vi "Sample.vi"(8 "Error In":errorcluster caption="错误输入", 10 "基本信息":T1={"USB Port"="COM1", "采集间隔(s)"=0.5, "压力设备选择"=TRUE}) -> (0 "Error Out":errorcluster caption="错误输出", 2 "Data":dbl[](array[numeric]))   [LabVIEW 2026, in "UI-压力.lvlib" / "Acquisition.lvlib"]
uses:
  Acquisition.lvlib
  Supports/Device Info.ctl
  <vilib>/Analysis/baseanly.llb/Mean (DBL).vi
  <vilib>/Analysis/NI_AALBase.lvlib
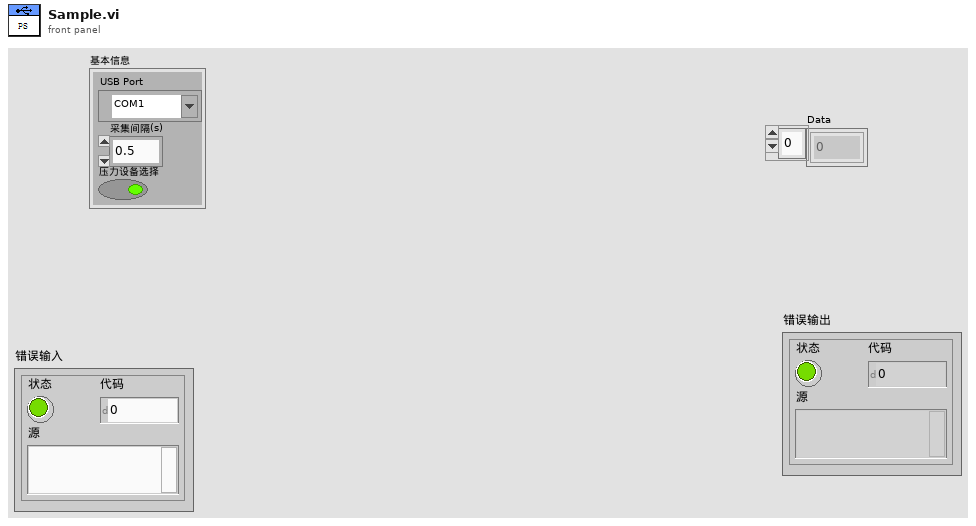
[diagram p1: front panel]
types:
  T1 = typedef "UI-压力.lvlib/Device Info.ctl" = cluster{"USB Port":refnum<visa-resource-name>, "采集间隔(s)":dbl, "压力设备选择":bool}
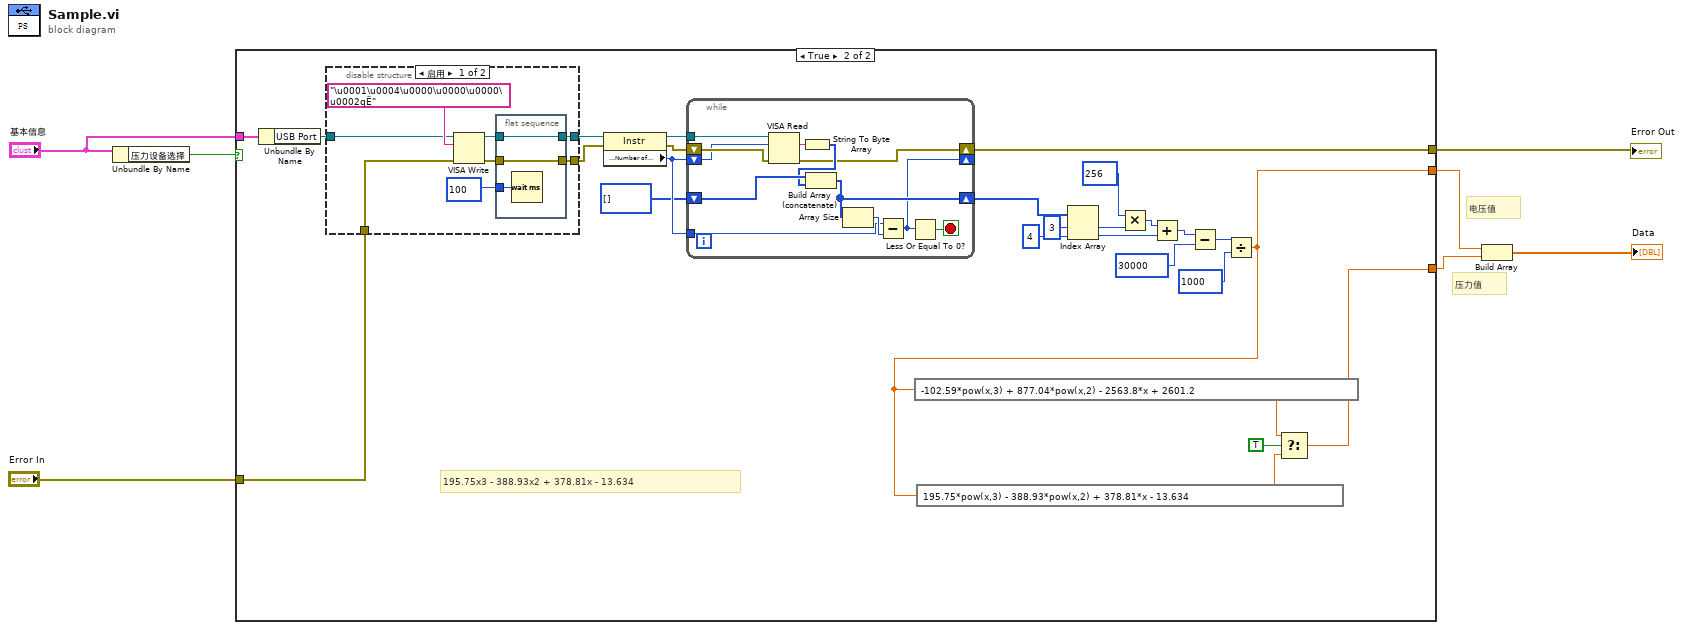
[diagram p0: block diagram]
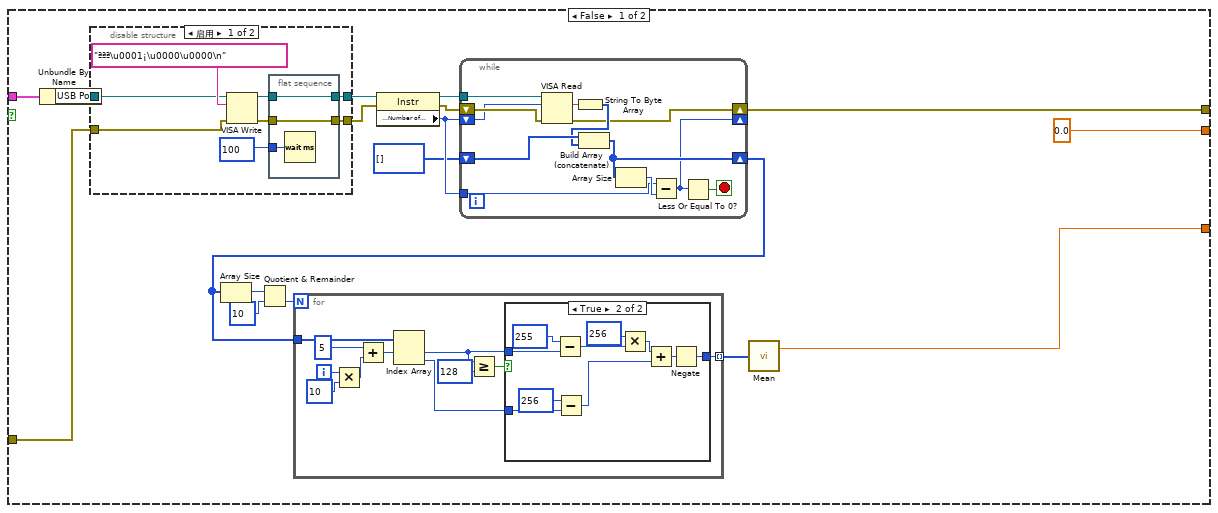
[diagram p2: hidden frame]
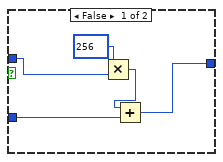
[diagram p4: hidden frame]
diagram:
  # "压力值"
  # "电压值"
  n1 = Unbundle By Name("基本信息") -> ("压力设备选择"=w7:bool)
  n2 = case shown="True" w7 {
    tunnel: [0.0 ("Scalar") w78] -> w5
    tunnel: "基本信息" -> [w20 w96]
    tunnel: [w11 w79] -> w4
    tunnel: "Error In" -> [w10 w77]
    tunnel: [w8 w75] -> w1
    frame False {
      n3 = Unbundle By Name(w20) -> ("USB Port"=w18:refnum<visa-resource-name>)
      n4 = disable-structure shown="启用" {
        disable-tunnel: w18 -> [w28 w36]
        disable-tunnel: [w27 w36] -> w17
        disable-tunnel: w10 -> [w26 _]
        disable-tunnel: [w25 _] -> w9
        frame Enabled {
          n5 = VISA Write(VISA resource name=w28, write buffer="ªªª\u0001¡\u0000\u0000\n" ("Command"), error in (no error)=w26) -> (VISA resource name out=w31:refnum<visa-resource-name>, error out=w32:errorcluster)  [unwired: 1 out]
          n6 = flat-sequence {
            tunnel: w32 -> [w34]
            tunnel: [w34] -> w25
            tunnel: w31 -> [w33]
            tunnel: [w33] -> w27
            tunnel: u32 100 ("读取前延时(ms)") -> [w35]
            frame #0 {
              n7 = Wait (ms)(milliseconds to wait=w35) -> ()  [unwired: 1 out]
            }
          }
        }
        frame Disabled {
        }
      }
      n8 = property class="Instr"(reference=w17, error in=w9) -> (reference out=w24:refnum<visa-resource-name>, error out=w23:errorcluster, "Serial Settings:Number of Bytes at Serial Port"=w22:u32)
      n9 = while {
        tunnel: w24 -> [w72]
        shift-right: [w74] -> w13
        shift-left: u8[] [] ("unsigned byte array") -> [w73]
        tunnel: w22 -> [w66]
        shift-right: [w64] -> _
        shift-left: w22 -> [w70]
        shift-right: [w63] -> w8
        shift-left: w23 -> [w71]
        stop <- w65 stop-if-true
        n10 = VISA Read(VISA resource name=w72, byte count=w70, error in (no error)=w71) -> (read buffer=w69:string, error out=w63:errorcluster)  [unwired: 2 out]
        n11 = String To Byte Array(string=w69) -> (unsigned byte array=w68:u8[])
        n12 = Build Array (concatenate)(w73, w68) -> (w74:u8[])
        n13 = Array Size(array=w74) -> (size(s)=w67:i32)
        n14 = Subtract(x=w66, y=w67) -> (x-y=w64:u32)
        n15 = Less Or Equal To 0?(x=w64) -> (x <= 0?=w65:bool)
      }
      n16 = Array Size(array=w13) -> (size(s)=w15:i32)
      n17 = Quotient & Remainder(x=w15, y=10) -> (floor(x/y)=w14:i32)  [unwired: 1 out]
      n18 = for {
        N: w14 -> [_]
        tunnel: w13 -> [w47]
        tunnel: [w37] -> w12 mode=indexing
        i -> [w44]
        n19 = Multiply(x=w44, y=10) -> (x*y=w42:i32)
        n20 = Add(x=5 ("索引"), y=w42) -> (x+y=w45:i32)
        n21 = Index Array(array=w47, index #1=w45) -> (element #1=w39:u8, element #2=w38:u8)  [unwired: 1 in]
        n22 = Greater Or Equal?(x=w39, y=128) -> (x >= y?=w41:bool)
        n23 = case shown="True" w41 {
          tunnel: w39 -> [w51 w60]
          tunnel: w38 -> [w49 w58]
          tunnel: [w48 w53] -> w37
          frame False {
            n24 = Multiply(x=256, y=w51) -> (x*y=w52:i32)
            n25 = Add(x=w52, y=w49) -> (x+y=w48:i32)
          }
          frame True {
            n26 = Subtract(x=255, y=w60) -> (x-y=w57:i32)
            n27 = Subtract(x=256, y=w58) -> (x-y=w55:i32)
            n28 = Multiply(x=256, y=w57) -> (x*y=w56:i32)
            n29 = Add(x=w56, y=w55) -> (x+y=w54:i32)
            n30 = Negate(x=w54) -> (-x=w53:i32)
          }
        }
      }
      n31 = call-poly <vilib>:"Mean.vi"("X"=w12) -> ("mean"=w11:dbl)  [unwired: 1 out]
    }
    frame True {
      # "195.75x3 - 388.93x2 + 378.81x - 13.634"
      n32 = Unbundle By Name(w96) -> ("USB Port"=w95:refnum<visa-resource-name>)
      n33 = disable-structure shown="启用" {
        disable-tunnel: w95 -> [w104 w112]
        disable-tunnel: [w103 w112] -> w94
        disable-tunnel: w77 -> [w102 _]
        disable-tunnel: [w101 _] -> w76
        frame Enabled {
          n34 = VISA Write(VISA resource name=w104, write buffer="\u0001\u0004\u0000\u0000\u0000\u0002qË" ("Command"), error in (no error)=w102) -> (VISA resource name out=w107:refnum<visa-resource-name>, error out=w108:errorcluster)  [unwired: 1 out]
          n35 = flat-sequence {
            tunnel: w108 -> [w110]
            tunnel: [w110] -> w101
            tunnel: w107 -> [w109]
            tunnel: [w109] -> w103
            tunnel: u32 100 ("读取前延时(ms)") -> [w111]
            frame #0 {
              n36 = Wait (ms)(milliseconds to wait=w111) -> ()  [unwired: 1 out]
            }
          }
        }
        frame Disabled {
        }
      }
      n37 = property class="Instr"(reference=w94, error in=w76) -> (reference out=w100:refnum<visa-resource-name>, error out=w99:errorcluster, "Serial Settings:Number of Bytes at Serial Port"=w98:u32)
      n38 = while {
        tunnel: w100 -> [w122]
        shift-right: [w124] -> w93
        shift-left: u8[] [] ("unsigned byte array") -> [w123]
        tunnel: w98 -> [w116]
        shift-right: [w114] -> _
        shift-left: w98 -> [w120]
        shift-right: [w113] -> w75
        shift-left: w99 -> [w121]
        stop <- w115 stop-if-true
        n39 = VISA Read(VISA resource name=w122, byte count=w120, error in (no error)=w121) -> (read buffer=w119:string, error out=w113:errorcluster)  [unwired: 2 out]
        n40 = String To Byte Array(string=w119) -> (unsigned byte array=w118:u8[])
        n41 = Build Array (concatenate)(w123, w118) -> (w124:u8[])
        n42 = Array Size(array=w124) -> (size(s)=w117:i32)
        n43 = Subtract(x=w116, y=w117) -> (x-y=w114:u32)
        n44 = Less Or Equal To 0?(x=w114) -> (x <= 0?=w115:bool)
      }
      n45 = Index Array(array=w93, index #1=3 ("索引"), index #2=4 ("索引")) -> (element #1=w92:u8, element #2=w91:u8)
      n46 = Multiply(x=u16 256, y=w92) -> (x*y=w90:u16)
      n47 = Add(x=w90, y=w91) -> (x+y=w89:u16)
      n48 = Subtract(x=w89, y=u16 30000) -> (x-y=w84:u16)
      n49 = Divide(x=w84, y=u16 1000) -> (x/y=w78:dbl)
      n50 = expression code="-102.59*pow(x,3) + 877.04*pow(x,2) - 2563.8*x + 2601.2"(w78) -> (w80:dbl)
      n51 = expression code="195.75*pow(x,3) - 388.93*pow(x,2) + 378.81*x - 13.634"(w78) -> (w81:dbl)
      n52 = Select(t=w80, s=TRUE, f=w81) -> (s? t:f=w79:dbl)
    }
  }
  "Error Out" <- w1
  n53 = Build Array(w5, w4) -> (→"Data":dbl[])
